vi "SaveUserEventsToDisk.vi"(8 "error in":errorcluster, 11 "concatenated string":string) -> (0 "error out":errorcluster)   [LabVIEW 2026, in "UserEventRecorder.lvlib"]
uses:
  UserEventRecorder.lvlib
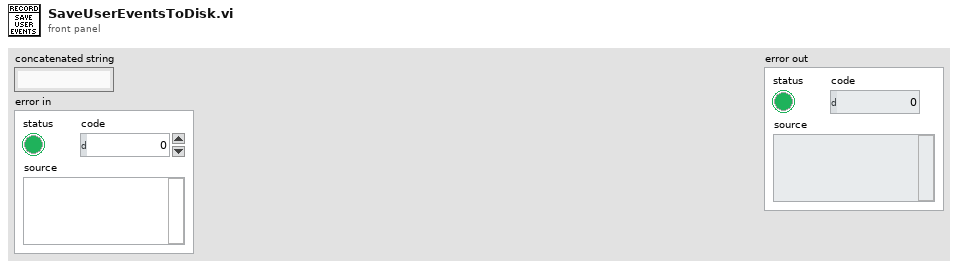
[diagram p1: front panel]
types:
  T1 = enum16{"open", "replace", "create", "open or create", "replace or create", "replace or create with confirmation"}
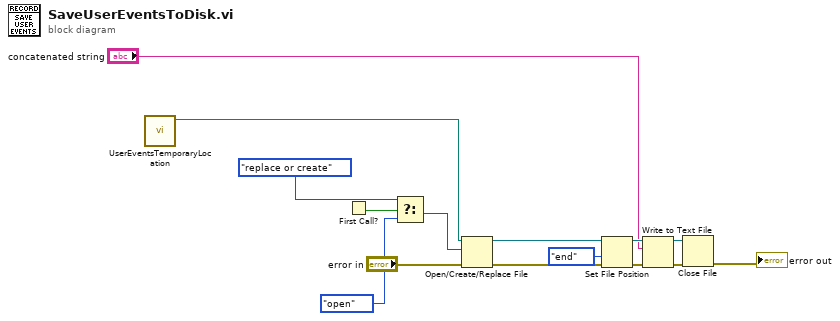
[diagram p0: block diagram]
diagram:
  n1 = call "UserEventsTemporaryLocation.vi"() -> ("UserEventsPath"=w4:path)  [unwired: 11 in]
  n2 = First Call?() -> (First Call?: T/F=w8:bool)
  n3 = Select(t=T1."replace or create" ("operation (0:open)"), s=w8, f=T1."open" ("operation (0:open)")) -> (s? t:f=w5:T1)
  n4 = Open/Create/Replace File(file path (use dialog)=w4, error in="error in", operation (0:open)=w5) -> (refnum out=w15:refnum<file>, error out=w14:errorcluster)  [unwired: 3 in, 1 out]
  n5 = Set File Position(refnum=w15, from (0:start)=enum16{"start", "end", "current"}."end", error in=w14) -> (refnum out=w12:refnum<file>, error out=w13:errorcluster)  [unwired: 1 in]
  n6 = Write to Text File(file (use dialog)=w12, text="concatenated string", error in=w13) -> (refnum out=w10:refnum<file>, error out=w9:errorcluster)  [unwired: 1 in, 1 out]
  n7 = Close File(refnum=w10, error in=w9) -> (error out=→"error out":errorcluster)  [unwired: 1 out]
